vi "libssh2_session_last_error.vi"(8 "error in (no error)":errorcluster, 11 "session":T1) -> (0 "error out":errorcluster, 1 "error message":string, 2 "error code":i32)   [LabVIEW 2017, in "libssh2.lvlib"]
doc: "Get the last error code and error message for a session."
uses:
  libssh2.lvlib
  Session Refnum.ctl
  Global Settings.vi
  Read Session Refnum.vi
  <vilib>/Utility/semaphor.llb/Acquire Semaphore.vi
  <vilib>/Utility/semaphor.llb/Release Semaphore.vi
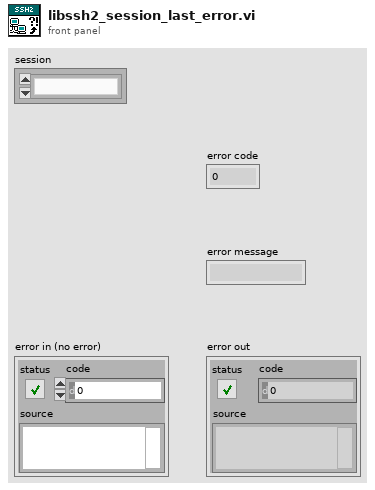
[diagram p1: front panel]
types:
  T1 = typedef "libssh2.lvlib/Session Refnum.ctl" = refnum<k1>
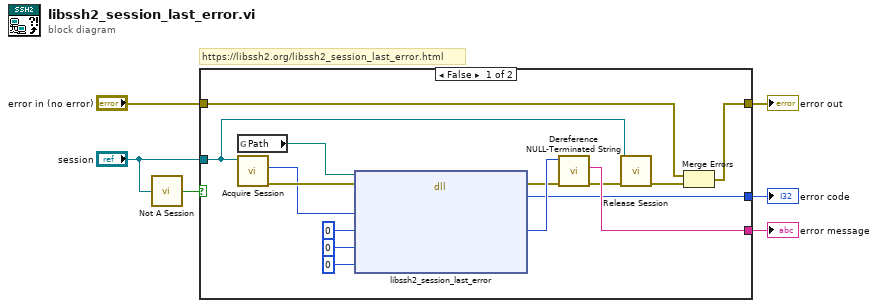
[diagram p0: block diagram]
diagram:
  # "https://libssh2.org/libssh2_session_last_error.html"
  n1 = call "Not A Session.vi"("session"="session") -> ("Not a Session?"=w1:bool)
  n2 = case shown="False" w1 {
    tunnel: [w12 w22] -> w6
    tunnel: [w17 _] -> w5
    tunnel: [w16 _] -> w4
    tunnel: "error in (no error)" -> [w13 w22]
    tunnel: "session" -> [w10 _]
    frame False {
      n3 = global read "Global Settings.vi" "Path"() -> (w11:path)
      n4 = call "Acquire Session.vi"("session"=w10) -> ("error out"=w15:errorcluster, "LIBSSH2_SESSION*"=w14:u64)  [unwired: 8 in, 1 out]
      n5 = dll-call lib="?" fn="libssh2_session_last_error"(path in=w11, error in=w15, "session"=w14, "errmsg"=u64 0, "errmsg_len"=0, "want_buf"=0) -> (error out=w9:errorcluster, "return value"=w16:i32, "errmsg"=w20:u64)  [unwired: 4 in, 1 out]
      n6 = call "Dereference NULL-Terminated String.vi"("error in (no error)"=w9, "char*"=w20) -> ("error out"=w8:errorcluster, "string"=w17:string)  [unwired: 8 in]
      n7 = call "Release Session.vi"("error in (no error)"=w8, "session"=w10) -> ("error out"=w7:errorcluster)  [unwired: 9 in]
      n8 = Merge Errors(w13, w7) -> (w12:errorcluster)
    }
    frame True {
    }
  }
  "error out" <- w6
  "error message" <- w5
  "error code" <- w4
